vi "RDC-get_dielectric.vi"(8 "dielectric":T1) -> (11 "speed of light C":dbl=300000000.0, 14 "er":dbl, 15 "sqrt(er)":dbl, 16 "tanQ":dbl, 18 "Vp":dbl, 19 "VF":dbl)   [LabVIEW 2020, in "RDC-Reflection_Data_Computation.lvlib"]
doc: "Returns the stored properties of the selected coax dielectric (Teflon or Eccostock 0005): er, sqrt(er), tanQ, Vp, VF and the speed of light constant."
uses:
  RDC-Reflection_Data_Computation.lvlib
  RDC-dielectric_types.ctl
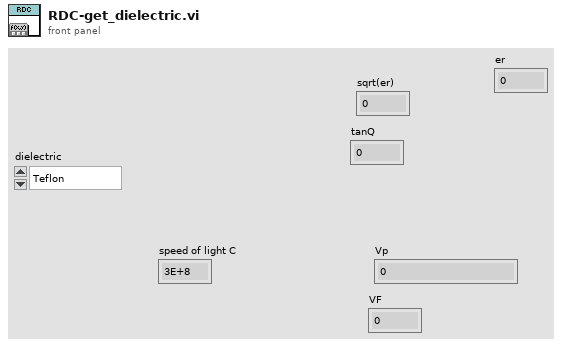
[diagram p1: front panel]
types:
  T1 = typedef "RDC-Reflection_Data_Computation.lvlib/RDC-dielectric_types.ctl" = enum16{"Teflon", "Eccostock 0005"}
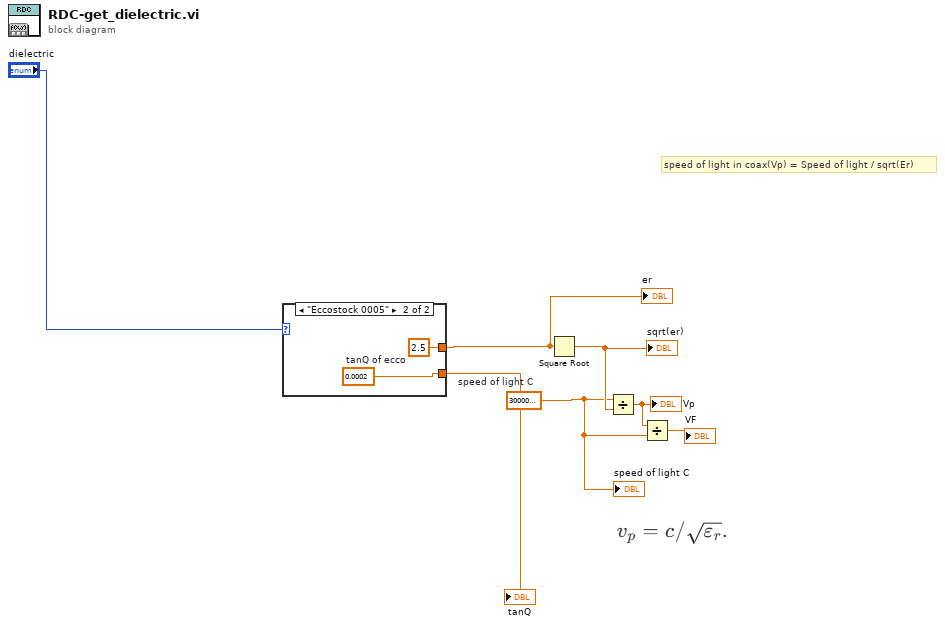
[diagram p0: block diagram]
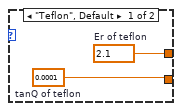
[diagram p2: hidden frame]
diagram:
  w3 = 300000000.0  # speed of light C
  # "speed of light in coax(Vp) = Speed of light / sqrt(Er)"
  n1 = case shown="\"Eccostock 0005\"" "dielectric" {
    tunnel: [w9 2.5 ("Er of teflon")] -> w5
    tunnel: [w8 w10] -> w1
    frame "Teflon", Default {
      w8 = 0.0001  # tanQ of teflon
      w9 = 2.1  # Er of teflon
    }
    frame "Eccostock 0005" {
      w10 = 0.0002  # tanQ of ecco
    }
  }
  "er" <- w5
  "tanQ" <- w1
  n2 = Square Root(x=w5) -> (sqrt(x)=w7:dbl)
  "sqrt(er)" <- w7
  n3 = Divide(x=w3, y=w7) -> (x/y=w4:dbl)
  "Vp" <- w4
  n4 = Divide(x=w4, y=w3) -> (x/y=→"VF":dbl)
  "speed of light C" <- w3
